vi "Byte to Bits.vi"(0 "Byte":u8 format="%02x", 7 "Bit Width":i32=8, 11 "error in (no error)":errorcluster) -> (4 "Bits":u8[](array[numeric]), 15 "error out":errorcluster)   [LabVIEW 2018, in "MIPI RFFE API.lvlib"]
uses:
  MIPI RFFE API.lvlib
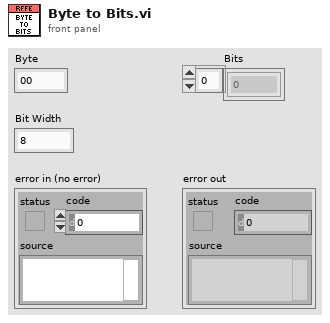
[diagram p1: front panel]
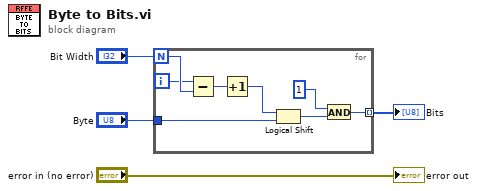
[diagram p0: block diagram]
diagram:
  n1 = for {
    N: "Bit Width" -> [w12]
    tunnel: "Byte" -> [w8]
    tunnel: [w5] -> w1 mode=indexing
    i -> [w11]
    n2 = Subtract(x=w11, y=w12) -> (x-y=w10:i32)
    n3 = Increment(x=w10) -> (x+1=w9:i32)
    n4 = Logical Shift(y=w9, x=w8) -> (x << y=w7:u8)
    n5 = And(x=u8 1, y=w7) -> (x .and. y?=w5:u8)
  }
  "Bits" <- w1
  "error out" <- "error in (no error)"
